vi "Close.vi"(8 "error in (no error)":errorcluster, 11 "Modbus_AI in":refnum<class "Modbus_AI.lvclass">) -> (0 "error out":errorcluster, 3 "Modbus_AI out":refnum<class "Modbus_AI.lvclass">)   [LabVIEW 2021, in "Modbus_AI.lvclass"]
uses:
  Modbus_AI.lvclass
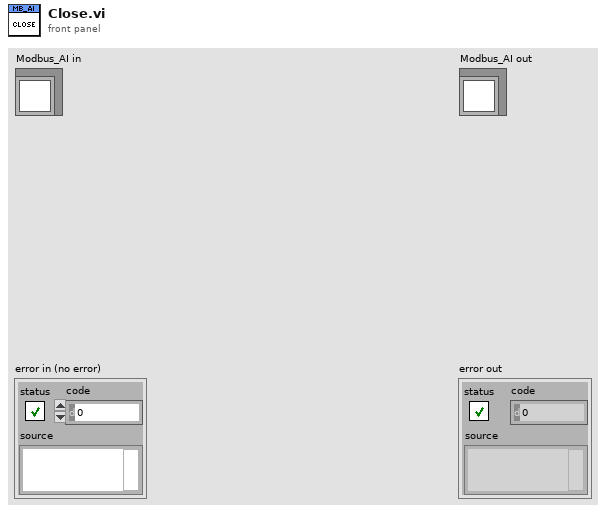
[diagram p1: front panel]
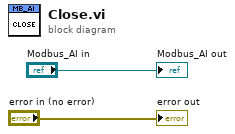
[diagram p0: block diagram]
diagram:
  "error out" <- "error in (no error)"
  "Modbus_AI out" <- "Modbus_AI in"
